vi "SMS Analysis Interface.vi"(7 "Calling VI Ref":refnum<vi>) -> ()   [LabVIEW 2016]
uses:
  <vilib>/Utility/miscctls.llb/LVPointTypeDef.ctl
  Orca Flash Data Spooler/Orca Data Spooler Type Defs/Orca Data Spooler Transfer Data.ctl
  SMS Analysis Interface Type Defs/SMS Analysis Interface Connection Info.ctl
panel:
  in  "Clear Queue":bool
  out "Connection Error":bool
  out "Remote Running":bool
  out "Remote Ready":bool
  in  "Queue List":i32(listbox)
  in  "Pause Queue":bool
  in  "Quit Remote":bool
  in  "Add Dataset":bool
  in  "Quit":bool
  out "Start Up Error":errorcluster
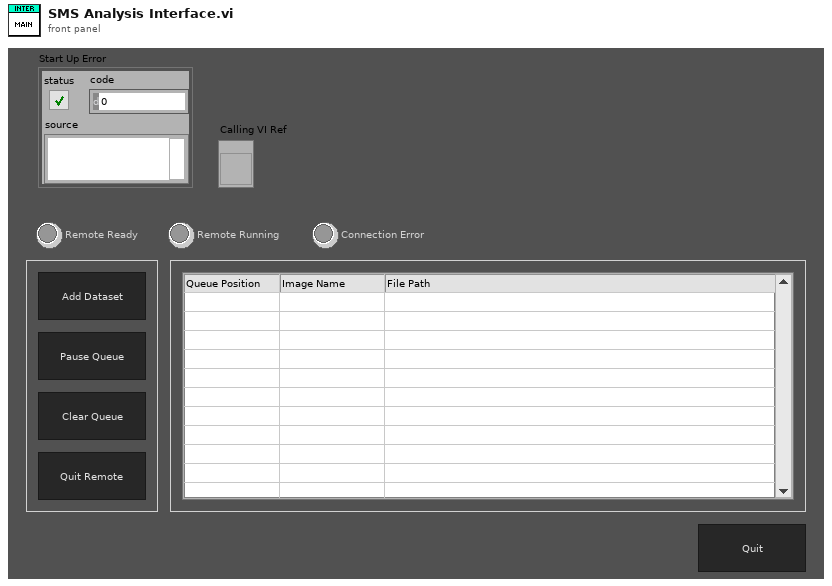
[diagram p1: front panel]
types:
  T1 = typedef "SMS Analysis Interface Connection Info.ctl" = cluster{"Remote IP":string, "Port":u16}
  T2 = typedef "Orca Data Spooler Transfer Data.ctl" = cluster{"transLogPath":string, "imageName":string, "noFrames":u32, "noCycles":u16, "quitFlag":bool, "channelCode":u8, "setupName":string}
  T3 = enum16{"Always On", "Always Off", "Off While Running"}
  T4 = typedef "LVPointTypeDef.ctl" = cluster{"Horizontal":i16, "Vertical":i16}
  T5 = typedef "LVRectTypeDef.ctl" = cluster{"Left":i16, "Top":i16, "Right":i16, "Bottom":i16}
  T6 = typedef "LVBoundsTypeDef.ctl" = cluster{"Width":u32, "Height":u32}
  T7 = enum32{"Bad", "Idle", "Run top level", "Running"}
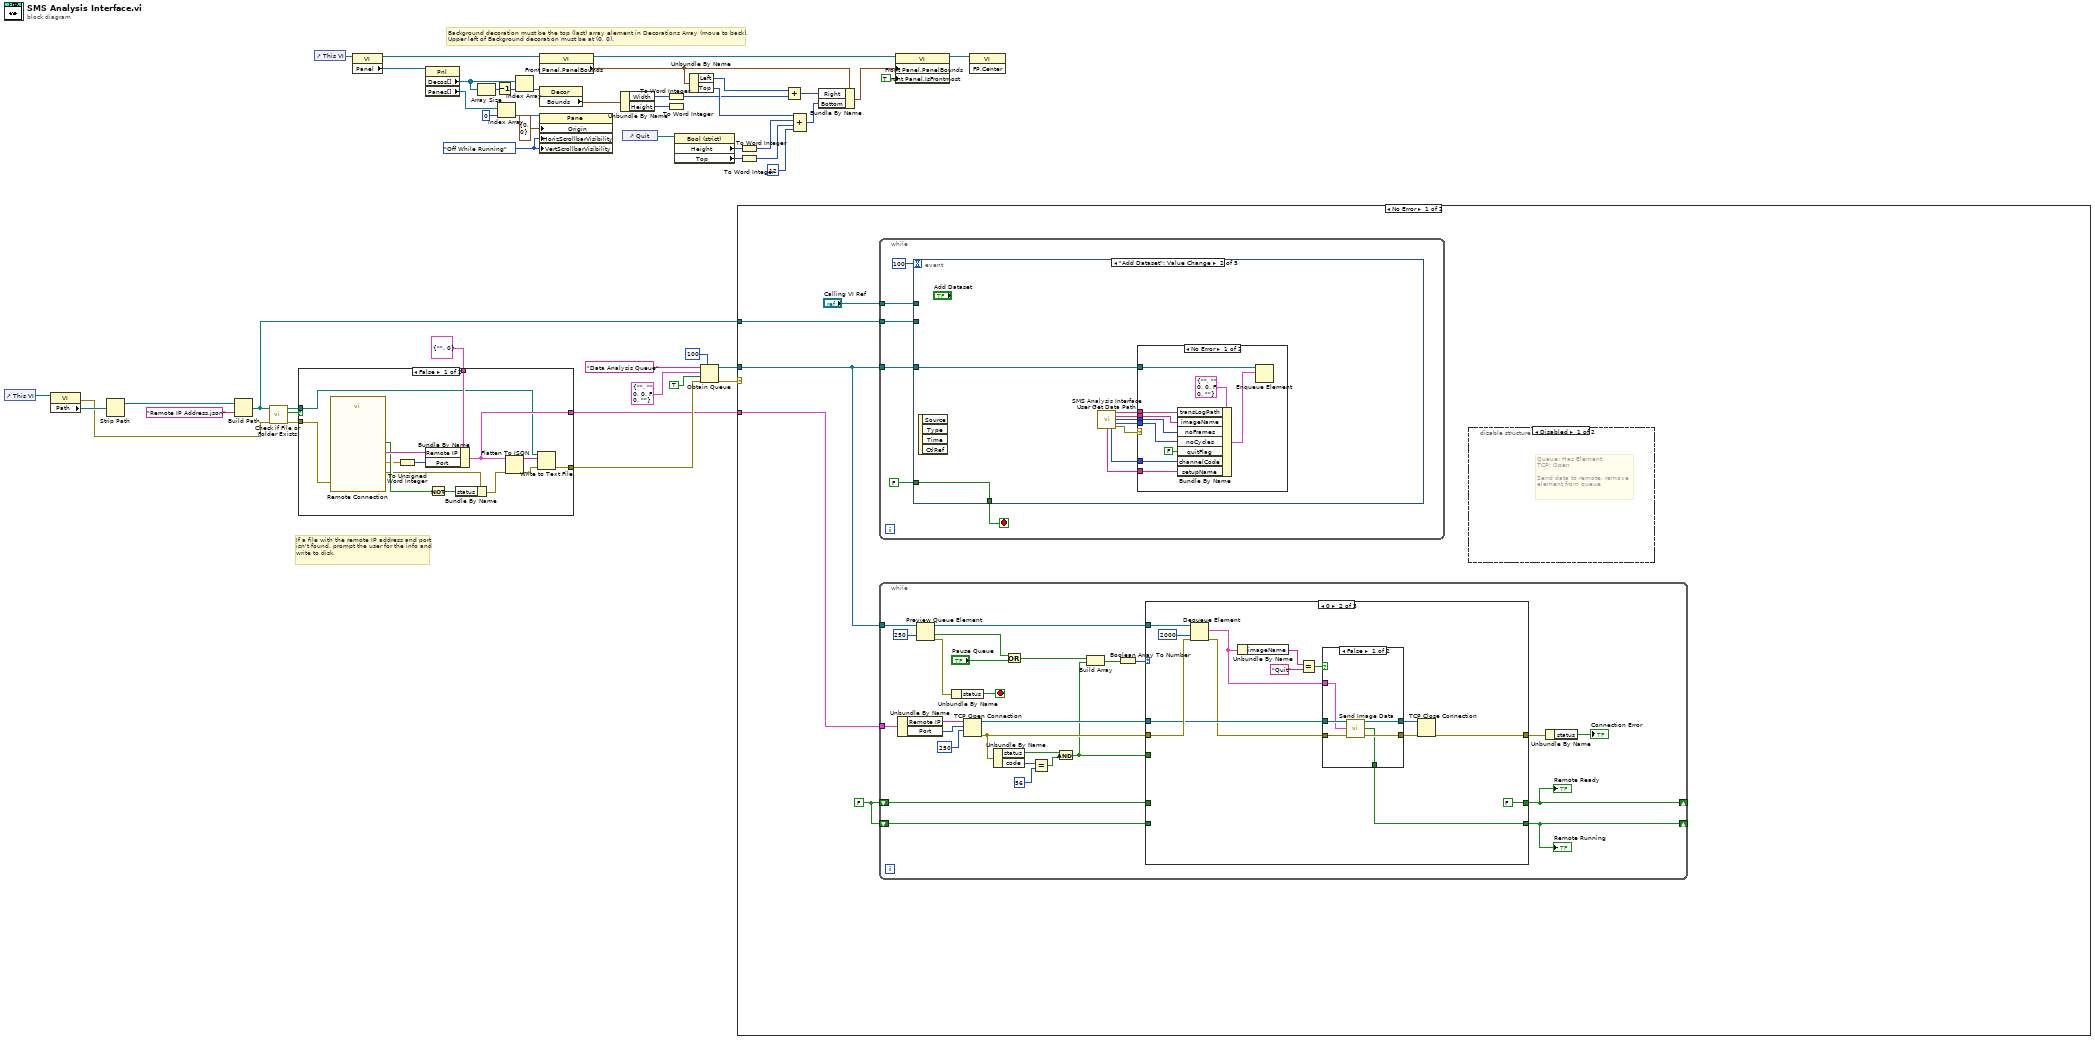
[diagram p0: block diagram]
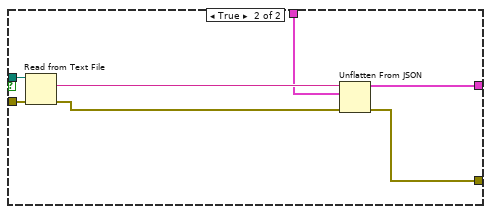
[diagram p2: hidden frame]
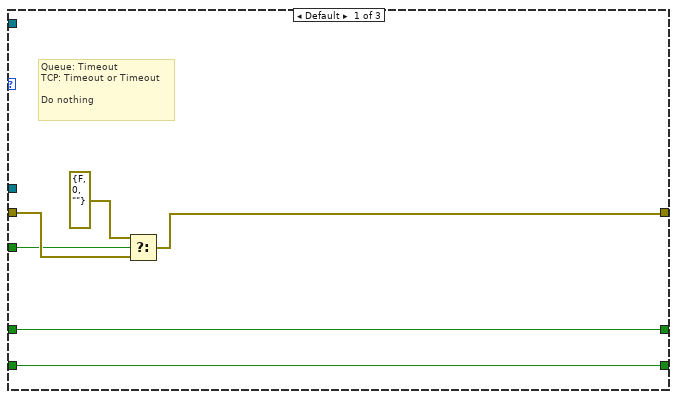
[diagram p4: hidden frame]
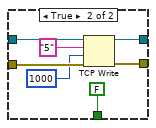
[diagram p5: hidden frame]
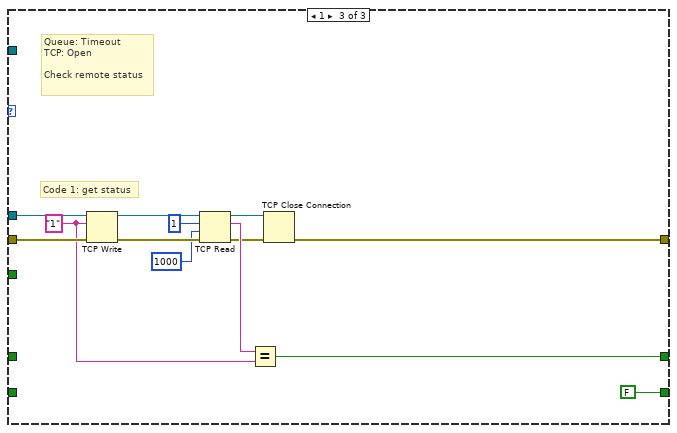
[diagram p6: hidden frame]
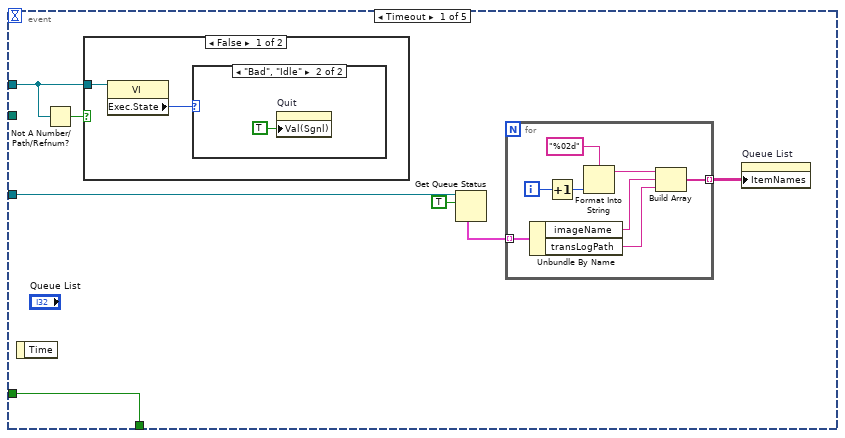
[diagram p7: hidden frame]
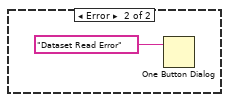
[diagram p10: hidden frame]
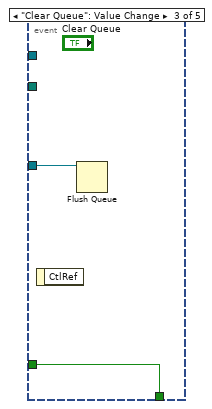
[diagram p11: hidden frame]
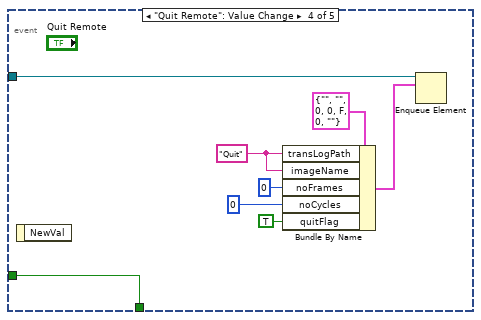
[diagram p12: hidden frame]
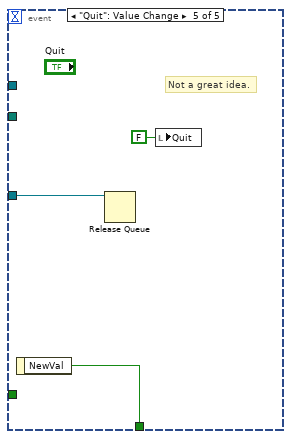
[diagram p13: hidden frame]
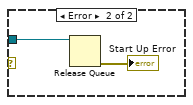
[diagram p14: hidden frame]
diagram:
  w26 = T3."Off While Running" ("Vertical Scrollbar Visibility")
  # "If a file with the remote IP address and port isn't found, prompt the user for the info and write to disk."
  # "Background decoration must be the top (last) array element in Decorations Array (move to back).\nUpper left of Background decoration must be at (0, 0)."
  n1 = control-ref of="This VI"() -> (w49:refnum<vi>)
  n2 = property class="VI"(reference=w49) -> (error out=w5:errorcluster, "Path"=w48:path)  [unwired: 1 in, 1 out]
  n3 = Strip Path(path=w48) -> (stripped path=w46:path)  [unwired: 1 out]
  n4 = Build Path(base path=w46, name or relative path="Remote IP Address.json" ("name (unnamed)")) -> (appended path=w14:path)
  n5 = call <vilib>:"Check if File or Folder Exists.vi"("error in (no error)"=w5, "path"=w14) -> ("error out"=w6:errorcluster, "file or folder exists?"=w44:bool, "dup path"=w45:path)  [unwired: 7 in]
  n6 = case shown="False" w44 {
    tunnel: w45 -> [w56 w68]
    tunnel: [w62 w67] -> w1
    tunnel: T1 {"Remote IP"="", "Port"=0} ("Connection Data") -> [w63 w66]
    tunnel: [w57 w64] -> w4
    tunnel: w6 -> [w54 w65]
    frame False {
      n7 = call "Remote Connection"("error in (no error)"=w54) -> ("Port"=w51:dbl, "IP Address"=w55:string, "OK"=w53:bool, "error out"=w52:errorcluster)  [unwired: 15 in]
      n8 = To Unsigned Word Integer(number=w51) -> (unsigned 16bit integer=w50:u16)
      n9 = Bundle By Name(cluster=w63, "Remote IP"=w55, "Port"=w50) -> (w62:T1)
      n10 = Not(x=w53) -> (.not. x?=w59:bool)
      n11 = Bundle By Name(cluster=w52, "status"=w59) -> (w58:errorcluster)
      n12 = Flatten To JSON(anything=w62, error in (no error)=w58) -> (JSON string=w61:string, 11:w60:errorcluster)  [unwired: 1 in]
      n13 = Write to Text File(file (use dialog)=w56, text=w61, error in=w60) -> (error out=w57:errorcluster)  [unwired: 1 in, 2 out]
    }
    frame True {
      n14 = Read from Text File(file (use dialog)=w68, error in=w65) -> (text=w70:string, error out=w69:errorcluster)  [unwired: 2 in, 2 out]
      n15 = Unflatten From JSON(JSON string=w70, type and defaults=w66, error in (no error)=w69) -> (value=w67:T1, error out=w64:errorcluster)  [unwired: 4 in]
    }
  }
  n16 = control-ref of="This VI"() -> (w18:refnum<vi>)
  n17 = property class="VI"(reference=w18) -> (reference out=w27:refnum<vi>, "Panel"=w19:refnum<vi>)  [unwired: 1 in, 1 out]
  n18 = property class="Pnl"(reference=w19) -> ("Decos[]"=w17:refnum<vi>[], "Panes[]"=w23:refnum<vi>[])  [unwired: 1 in, 2 out]
  n19 = Array Size(array=w17) -> (size(s)=w15:i32)
  n20 = Decrement(x=w15) -> (x-1=w16:i32)
  n21 = Index Array(array=w23, index=0) -> (element=w22:refnum<vi>)
  n22 = Index Array(array=w17, index=w16) -> (element=w25:refnum<vi>)
  n23 = property class="VI"(reference=w27) -> (reference out=w29:refnum<vi>, "Front Panel.PanelBounds"=w30:T5)  [unwired: 1 in, 1 out]
  n24 = property class="Decor"(reference=w25) -> ("Bounds"=w28:T6)  [unwired: 1 in, 2 out]
  n25 = property class="Pane"(reference=w22, "Origin"=T4 {"Horizontal"=0, "Vertical"=0}, "HorizScrollbarVisibility"=w26, "VertScrollbarVisibility"=w26) -> ()  [unwired: 1 in, 2 out]
  n26 = Unbundle By Name(w28) -> ("Width"=w33:u32, "Height"=w36:u32)
  n27 = control-ref of="Quit"() -> (w20:refnum<vi>)
  n28 = To Word Integer(number=w33) -> (16bit integer=w35:i16)
  n29 = To Word Integer(number=w36) -> ()  [unwired: 1 out]
  n30 = property class="Bool (strict)"(reference=w20) -> ("Height"=w38:u32, "Top"=w39:i32)  [unwired: 1 in, 2 out]
  n31 = Unbundle By Name(w30) -> ("Left"=w32:i16, "Top"=w43:i16)
  n32 = Obtain Queue(max queue size (-1, unlimited)=100, name (unnamed)="Data Analysis Queue", element data type=T2 {"transLogPath"="", "imageName"="", "noFrames"=0, "noCycles"=0, "quitFlag"=FALSE, "channelCode"=0, "setupName"=""} ("Spooler Connection Data"), create if not found? (T)=TRUE, error in (no error)=w4) -> (queue out=w9:refnum<queue>, error out=w8:errorcluster)  [unwired: 1 out]
  n33 = case shown="No Error" w8 {
    tunnel: w14 -> [w75 _]
    tunnel: w9 -> [w74 w207]
    tunnel: w1 -> [w73 _]
    frame No Error {
      w72 = FALSE
      n34 = while {
        tunnel: w75 -> [w151]
        tunnel: w74 -> [w150]
        tunnel: "Calling VI Ref" -> [w149]
        stop <- w153 stop-if-true
        n35 = event shown="[1] \"Add Dataset\": Value Change" {
          selector: _ -> [_ _ _ _ _]
          dyn-events: _ -> [_ _ _ _ _]
          timeout: 100 -> [_ _ _ _ _]
          tunnel: FALSE -> [w161 w181 w194 w202 _]
          tunnel: [w161 w181 w194 w202 w205] -> w153
          tunnel: w151 -> [_ _ _ _ _]
          tunnel: w150 -> [w160 w180 w193 w195 w204]
          tunnel: w149 -> [w155 _ _ _ _]
          event Timeout {
            n36 = event-data() -> ()  [unwired: 1 in, 1 out]
            n37 = Not A Number/Path/Refnum?(number/path/refnum=w155) -> (NaN/Path/Refnum?=w156:bool)
            n38 = case shown="False" w156 {
              tunnel: w155 -> [w163 _]
              frame False {
                n39 = property class="VI"(reference=w163) -> ("Exec.State"=w162:T7)  [unwired: 1 in, 2 out]
                n40 = case shown="\"Bad\", \"Idle\"" w162 {
                  frame Default {
                  }
                  frame "Bad", "Idle" {
                    n41 = property on="Quit" class="Bool (strict)"("Val(Sgnl)"=TRUE ("Value (Signaling)")) -> ()  [unwired: 2 in, 2 out]
                  }
                }
              }
              frame True {
              }
            }
            n42 = Get Queue Status(queue=w160, return elements? (F)=TRUE) -> (elements=w159:T2[])  [unwired: 1 in, 7 out]
            n43 = for {
              tunnel: w159 -> [w172] mode=indexing
              tunnel: [w166] -> w157 mode=indexing
              i -> [w170]
              n44 = Unbundle By Name(w172) -> ("imageName"=w168:string, "transLogPath"=w167:string)
              n45 = Increment(x=w170) -> (x+1=w165:i32)
              n46 = Format Into String(format string="%02d", w165) -> (resulting string=w169:string)  [unwired: 2 in, 1 out]
              n47 = Build Array(w169, w168, w167) -> (w166:string[])
            }
            n48 = property on="Queue List" class="MCListbox (strict)"("ItemNames"=w157) -> ()  [unwired: 2 in, 2 out]
          }
          event "Add Dataset": Value Change {
            n49 = event-data() -> ()  [unwired: 1 in, 4 out]
            n50 = call "SMS Analysis Interface User Get Data Path.vi"() -> ("Transfer Log Path"=w179:string, "Image Name"=w178:string, "Frames"=w177:u32, "Cycles"=w176:u16, "setupName"=w173:string, "channelCode"=w174:u8, "Error"=w175:errorcluster)  [unwired: 9 in]
            n51 = case shown="No Error" w175 {
              tunnel: w180 -> [w189 _]
              tunnel: w179 -> [w187 _]
              tunnel: w178 -> [w186 _]
              tunnel: w177 -> [w185 _]
              tunnel: w176 -> [w184 _]
              tunnel: w174 -> [w183 _]
              tunnel: w173 -> [w182 _]
              frame No Error {
                n52 = Bundle By Name(cluster=T2 {"transLogPath"="", "imageName"="", "noFrames"=0, "noCycles"=0, "quitFlag"=FALSE, "channelCode"=0, "setupName"=""} ("Spooler Connection Data"), "transLogPath"=w187, "imageName"=w186, "noFrames"=w185, "noCycles"=w184, "quitFlag"=FALSE, "channelCode"=w183, "setupName"=w182) -> (w188:T2)
                n53 = Enqueue Element(queue=w189, element=w188) -> ()  [unwired: 2 in, 3 out]
              }
              frame Error {
                n54 = One Button Dialog(message="Dataset Read Error") -> ()  [unwired: 1 in, 1 out]
              }
            }
          }
          event "Clear Queue": Value Change {
            n55 = event-data() -> ()  [unwired: 1 in, 1 out]
            n56 = Flush Queue(queue=w193) -> ()  [unwired: 1 in, 3 out]
          }
          event "Quit Remote": Value Change {
            w196 = "Quit" ("transLogPath")
            n57 = event-data() -> ()  [unwired: 1 in, 1 out]
            n58 = Bundle By Name(cluster=T2 {"transLogPath"="", "imageName"="", "noFrames"=0, "noCycles"=0, "quitFlag"=FALSE, "channelCode"=0, "setupName"=""} ("Spooler Connection Data"), "transLogPath"=w196, "imageName"=w196, "noFrames"=u32 0, "noCycles"=u16 0, "quitFlag"=TRUE) -> (w199:T2)
            n59 = Enqueue Element(queue=w195, element=w199) -> ()  [unwired: 2 in, 3 out]
          }
          event "Quit": Value Change {
            # "Not a great idea."
            n60 = event-data() -> ("NewVal"=w205:bool)  [unwired: 1 in]
            n61 = Release Queue(queue=w204) -> ()  [unwired: 2 in, 3 out]
            n62 = local write "Quit"(FALSE ("Quit")) -> ()
          }
        }
      }
      n63 = while {
        tunnel: w74 -> [w102]
        tunnel: w73 -> [w98]
        shift-right: [w78] -> _
        shift-left: w72 -> [w81]
        shift-right: [w79] -> _
        shift-left: w72 -> [w80]
        stop <- w99 stop-if-true
        n64 = Unbundle By Name(w98) -> ("Remote IP"=w97:string, "Port"=w96:u16)
        n65 = Preview Queue Element(queue=w102, timeout in ms (-1)=250) -> (queue out=w85:refnum<queue>, timed out?=w95:bool, error out=w100:errorcluster)  [unwired: 1 in, 1 out]
        n66 = Unbundle By Name(w100) -> ("status"=w99:bool)
        n67 = TCP Open Connection(address=w97, remote port or service name=w96, timeout ms (60000)=250) -> (connection ID=w87:refnum<k5>, error out=w86:errorcluster)  [unwired: 2 in]
        n68 = Unbundle By Name(w86) -> ("status"=w89:bool, "code"=w92:i32)
        n69 = Or(x=w95, y="Pause Queue") -> (x .or. y?=w84:bool)
        n70 = Equal?(x=w92, y=56) -> (x = y?=w88:bool)
        n71 = And(x=w89, y=w88) -> (x .and. y?=w76:bool)
        n72 = Build Array(w84, w76) -> (w83:bool[])
        n73 = Boolean Array To Number(Boolean array=w83) -> (number=w82:u32)
        n74 = case shown="0" w82 {
          tunnel: w87 -> [_ w114 w148]
          tunnel: w86 -> [w107 w121 w144]
          tunnel: [w105 w118 w140] -> w77
          tunnel: w85 -> [_ w122 _]
          tunnel: w81 -> [w103 _ _]
          tunnel: w80 -> [w108 _ _]
          tunnel: [w103 FALSE w142] -> w78
          tunnel: [w108 w109 FALSE] -> w79
          tunnel: w76 -> [w104 _ _]
          frame Default {
            # "Queue: Timeout\nTCP: Timeout or Timeout\n\nDo nothing"
            n75 = Select(t=errorcluster {"status"=FALSE, "code"=0, "source"=""} ("error out"), s=w104, f=w107) -> (s? t:f=w105:errorcluster)
          }
          frame 0 {
            n76 = Dequeue Element(queue=w122, timeout in ms (-1)=2000, error in (no error)=w121) -> (element=w110:T2, error out=w113:errorcluster)  [unwired: 2 out]
            n77 = Unbundle By Name(w110) -> ("imageName"=w116:string)
            n78 = Equal?(x=w116, y="Quit") -> (x = y?=w115:bool)
            n79 = case shown="False" w115 {
              tunnel: w114 -> [w128 w134]
              tunnel: w113 -> [w127 w133]
              tunnel: [w126 w131] -> w112
              tunnel: [w125 w130] -> w111
              tunnel: w110 -> [w123 _]
              tunnel: [w124 FALSE ("Success")] -> w109
              frame False {
                n80 = call "Send Image Data.vi"("Connection In"=w128, "Image Data"=w123, "Error In"=w127) -> ("Connection Out"=w126:refnum<k5>, "Success"=w124:bool, "Error Out"=w125:errorcluster)  [unwired: 10 in]
              }
              frame True {
                n81 = TCP Write(connection ID=w134, data in="5", error in (no error)=w133, 9:1000 ("timeout ms (25000)")) -> (connection ID out=w131:refnum<k5>, error out=w130:errorcluster)  [unwired: 1 out]
              }
            }
            n82 = TCP Close Connection(connection ID=w112, error in (no error)=w111) -> (error out=w118:errorcluster)  [unwired: 1 in, 1 out]
          }
          frame 1 {
            w138 = "1" ("data in")
            # "Code 1: get status"
            # "Queue: Timeout\nTCP: Open\n\nCheck remote status"
            n83 = TCP Write(connection ID=w148, data in=w138, error in (no error)=w144) -> (connection ID out=w147:refnum<k5>, error out=w145:errorcluster)  [unwired: 1 in, 1 out]
            n84 = TCP Read(connection ID=w147, bytes to read=1, error in (no error)=w145, 9:1000 ("timeout ms (25000)")) -> (connection ID out=w136:refnum<k5>, data out=w139:string, error out=w137:errorcluster)  [unwired: 1 in]
            n85 = Equal?(x=w139, y=w138) -> (x = y?=w142:bool)
            n86 = TCP Close Connection(connection ID=w136, error in (no error)=w137) -> (error out=w140:errorcluster)  [unwired: 1 in, 1 out]
          }
        }
        "Remote Ready" <- w78
        "Remote Running" <- w79
        n87 = Unbundle By Name(w77) -> ("status"=→"Connection Error":bool)
      }
      n88 = disable-structure shown="Disabled" {
        frame Disabled {
          # "Queue: Has Element\nTCP: Open\n\nSend data to remote, remove element from queue"
        }
        frame Enabled {
        }
      }
    }
    frame Error {
      n89 = Release Queue(queue=w207) -> (error out=→"Start Up Error":errorcluster)  [unwired: 2 in, 2 out]
    }
  }
  n90 = To Word Integer(number=w38) -> (16bit integer=w41:i16)
  n91 = To Word Integer(number=w39) -> (16bit integer=w42:i16)
  n92 = Add(x=w32, y=w35) -> (x+y=w34:i16)
  n93 = Compound Arithmetic op=ADD(w43, w41, w42, i16 12 ("y")) -> (w37:i16)
  n94 = Bundle By Name(cluster=w30, "Right"=w34, "Bottom"=w37) -> (w31:T5)
  n95 = property class="VI"(reference=w29, "Front Panel.PanelBounds"=w31, "Front Panel.IsFrontmost"=TRUE ("Front Panel Window:Is Frontmost")) -> (reference out=w3:refnum<vi>)  [unwired: 1 in, 1 out]
  n96 = invoke class="VI" method="FP.Center"(reference=w3) -> ()  [unwired: 2 in, 3 out]
